vi "test tool error result.vi"(8 "error in (no error)":errorcluster) -> (0 "error out":errorcluster, 3 "body":string)   [LabVIEW 2020, in "MCP Server tests.lvlib"]
doc: "If the tool VI ran and its own error out has status true, the result of tools/call has isError true. The content still holds everything the tool returned. A tool whose error out has status false gets no isError."
uses:
  MCP Server tests.lvlib
  <vilib>/JDP Science/JSONtext/Next JSON Value.vi
  <vilib>/JDP Science/JSONtext/String Subset.vi
  <vilib>/JDP Science/JSONtext/Parsing/Advance past next JSON Value (inlined COPY).vi
  <vilib>/JDP Science/JSONtext/Parsing/Advance past whitespace.vi
  <vilib>/JDP Science/JSONtext/Parsing/Advance past String.vi
  <vilib>/JDP Science/JSONtext/Parsing/Advance past Number.vi
  <vilib>/JDP Science/JSONtext/Parsing/Advance past Line Ending.vi
  <vilib>/JDP Science/JSONtext/Parsing/Parse Full Path or Item Name.vi
  <vilib>/JDP Science/JSONtext/Parsing/Advance past Array.vi
  <vilib>/JDP Science/JSONtext/Parsing/Advance past Object.vi
  <vilib>/JDP Science/JSONtext/support/Error Cluster From Code.vi
  <vilib>/JDP Science/JSONtext/Offset/Find Item Locations by Path.vi
  <vilib>/addons/_JKI Toolkits/Caraya/classes/Test/Test.lvclass
  <vilib>/JDP Science/JSONtext/JSONtext.lvlib
  <vilib>/addons/_JKI Toolkits/Caraya/classes/Assert/Assert.lvclass
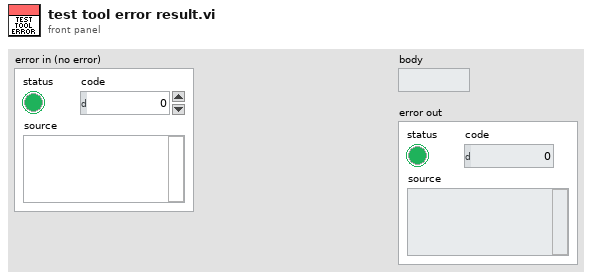
[diagram p1: front panel]
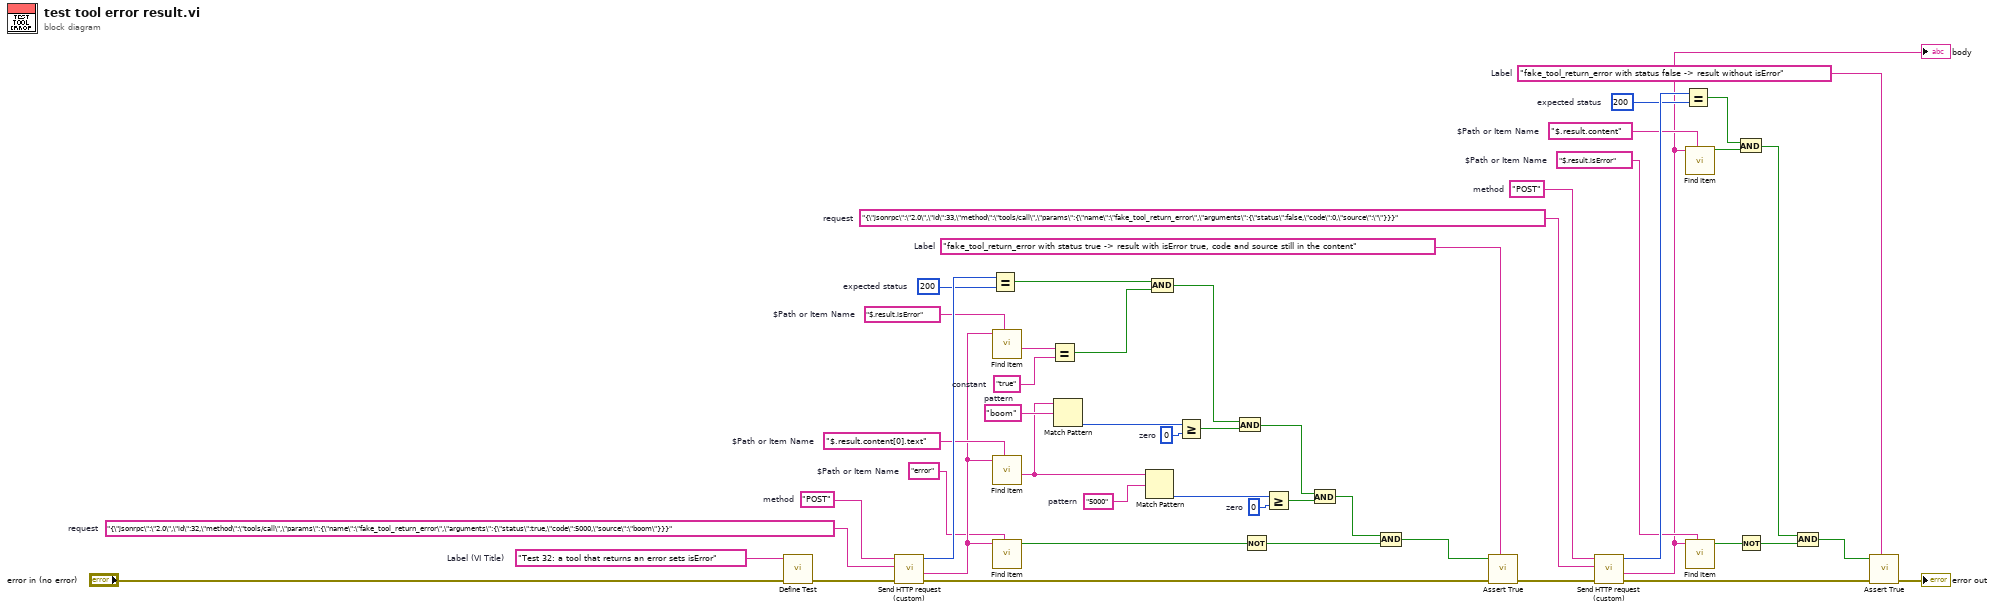
[diagram p0: block diagram]
diagram:
  w3 = "fake_tool_return_error with status false -> result without isError"  # Label
  w11 = "$.result.content"  # $Path or Item Name
  w12 = "$.result.isError"  # $Path or Item Name
  w13 = 200  # expected status
  w16 = "{\"jsonrpc\":\"2.0\",\"id\":33,\"method\":\"tools/call\",\"params\":{\"name\":\"fake_tool_return_error\",\"arguments\":{\"status\":false,\"code\":0,\"source\":\"\"}}}"  # request
  w17 = "POST"  # method
  w18 = "fake_tool_return_error with status true -> result with isError true, code and source still in the content"  # Label
  w30 = 0  # zero
  w32 = "5000"  # pattern
  w34 = 0  # zero
  w36 = "boom"  # pattern
  w37 = "true"  # constant
  w39 = "error"  # $Path or Item Name
  w41 = "$.result.content[0].text"  # $Path or Item Name
  w42 = "$.result.isError"  # $Path or Item Name
  w43 = 200  # expected status
  w46 = "{\"jsonrpc\":\"2.0\",\"id\":32,\"method\":\"tools/call\",\"params\":{\"name\":\"fake_tool_return_error\",\"arguments\":{\"status\":true,\"code\":5000,\"source\":\"boom\"}}}"  # request
  w47 = "POST"  # method
  w49 = "Test 32: a tool that returns an error sets isError"  # Label (VI Title)
  n1 = call <vilib>:"Define Test.vi"("error in (no error)"="error in (no error)", "Label (VI Title)"=w49) -> ("error out"=w45:errorcluster)  [unwired: 8 in, 1 out]
  n2 = call "Send HTTP request (custom).vi"("error in (no error)"=w45, "request"=w46, "method"=w47) -> ("error out"=w19:errorcluster, "response"=w40:string, "status code"=w44:i32)  [unwired: 5 in, 1 out]
  n3 = Equal?(x=w44, y=w43) -> (x = y?=w28:bool)
  n4 = call <vilib>:"Find Item.vi"("$Path or Item Name"=w42, "JSON"=w40) -> ("<JSON>"=w38:string)  [unwired: 6 in, 3 out]
  n5 = call <vilib>:"Find Item.vi"("$Path or Item Name"=w41, "JSON"=w40) -> ("<JSON>"=w33:string)  [unwired: 6 in, 3 out]
  n6 = call <vilib>:"Find Item.vi"("$Path or Item Name"=w39, "JSON"=w40) -> ("Found"=w29:bool)  [unwired: 6 in, 3 out]
  n7 = Equal?(x=w38, y=w37) -> (x = y?=w27:bool)
  n8 = Match Pattern(string=w33, regular expression=w36) -> (offset past match=w35:i32)  [unwired: 1 in, 3 out]
  n9 = Match Pattern(string=w33, regular expression=w32) -> (offset past match=w31:i32)  [unwired: 1 in, 3 out]
  n10 = And(x=w28, y=w27) -> (x .and. y?=w26:bool)
  n11 = Greater Or Equal?(x=w35, y=w34) -> (x >= y?=w25:bool)
  n12 = And(x=w26, y=w25) -> (x .and. y?=w24:bool)
  n13 = Not(x=w29) -> (.not. x?=w21:bool)
  n14 = Greater Or Equal?(x=w31, y=w30) -> (x >= y?=w23:bool)
  n15 = And(x=w24, y=w23) -> (x .and. y?=w22:bool)
  n16 = And(x=w22, y=w21) -> (x .and. y?=w20:bool)
  n17 = call <vilib>:"Assert True.vi"("Label"=w18, "error in (no error)"=w19, "True?"=w20) -> ("error out"=w15:errorcluster)  [unwired: 7 in, 1 out]
  n18 = call "Send HTTP request (custom).vi"("error in (no error)"=w15, "request"=w16, "method"=w17) -> ("error out"=w4:errorcluster, "response"=w2:string, "status code"=w14:i32)  [unwired: 5 in, 1 out]
  "body" <- w2
  n19 = Equal?(x=w14, y=w13) -> (x = y?=w9:bool)
  n20 = call <vilib>:"Find Item.vi"("$Path or Item Name"=w11, "JSON"=w2) -> ("Found"=w8:bool)  [unwired: 6 in, 3 out]
  n21 = call <vilib>:"Find Item.vi"("$Path or Item Name"=w12, "JSON"=w2) -> ("Found"=w10:bool)  [unwired: 6 in, 3 out]
  n22 = And(x=w9, y=w8) -> (x .and. y?=w7:bool)
  n23 = Not(x=w10) -> (.not. x?=w6:bool)
  n24 = And(x=w7, y=w6) -> (x .and. y?=w5:bool)
  n25 = call <vilib>:"Assert True.vi"("Label"=w3, "error in (no error)"=w4, "True?"=w5) -> ("error out"=→"error out":errorcluster)  [unwired: 7 in, 1 out]
